vi "Main.vi"() -> ()   [LabVIEW 2026]
doc: "Use this template to build a simple state machine design pattern. Each state executes code and determines which state to transition to."
uses:
  controls/Data.ctl
  controls/State.ctl
panel:
  out "Pos":i32(slide) scale=0.0..250.0
  out "Level 2":bool
  out "Level 1":bool
  out "going up":bool
  out "going down":bool
  out "Up":bool
  out "Down":bool
  in  "Stop":bool
  in  "Up":bool
  in  "Down":bool
  in  "Data":T1
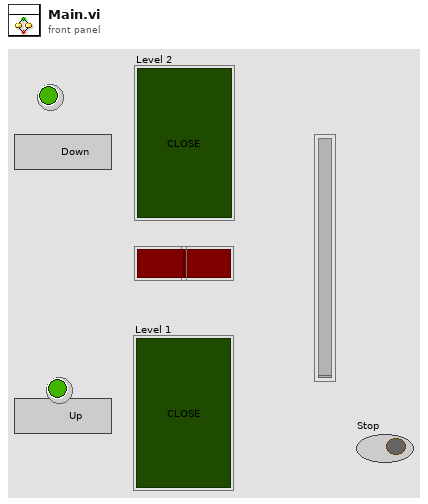
[diagram p1: front panel]
types:
  T1 = typedef "Data.ctl" = cluster{"Level":i32, "Down Pressed":bool, "Up Pressed\n":bool, "Moving Down\n":bool, "Moving Up\n":bool, "L1 Door Open":bool, "L2 Door Open":bool, "Counter":i32, "Previous State":T2, "Pos":i32}
  T2 = typedef "State.ctl" = enum16{"Initialize", "Wait for Event", "Open/Close L1", "Open/Close L2", "Moving Down", "Moving Up", "Exit", ""}
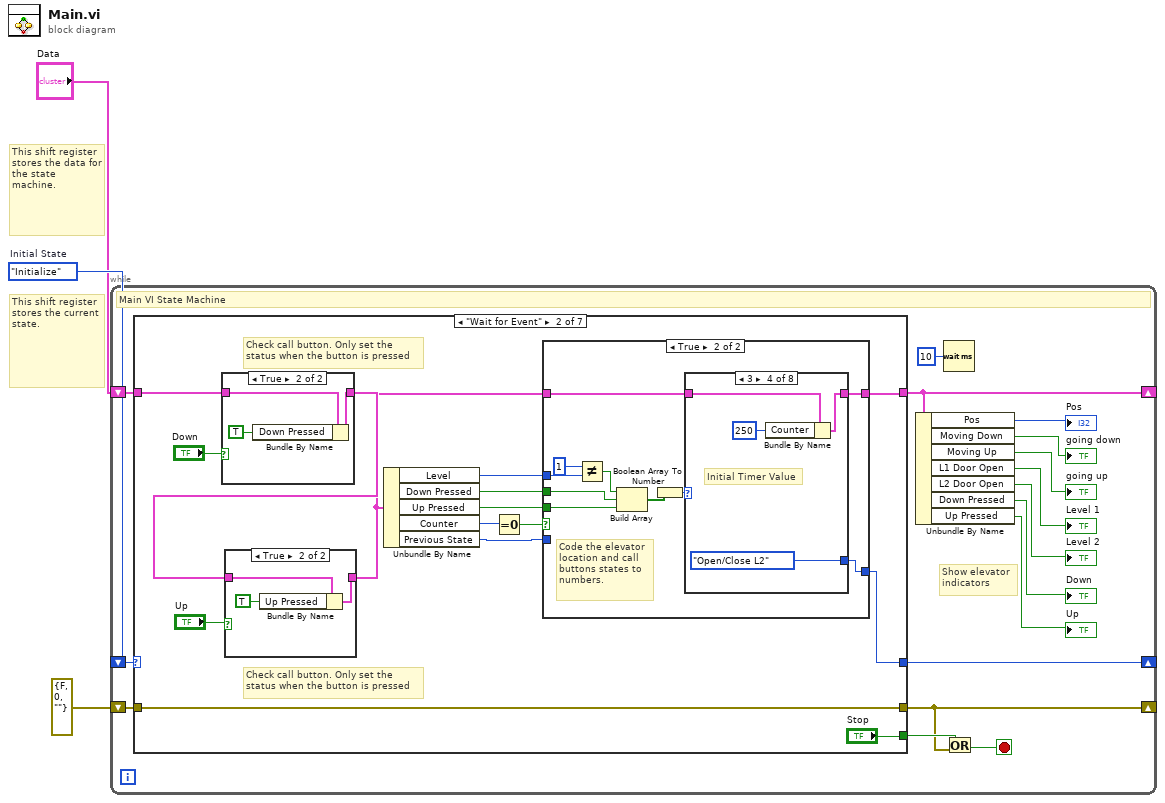
[diagram p0: block diagram]
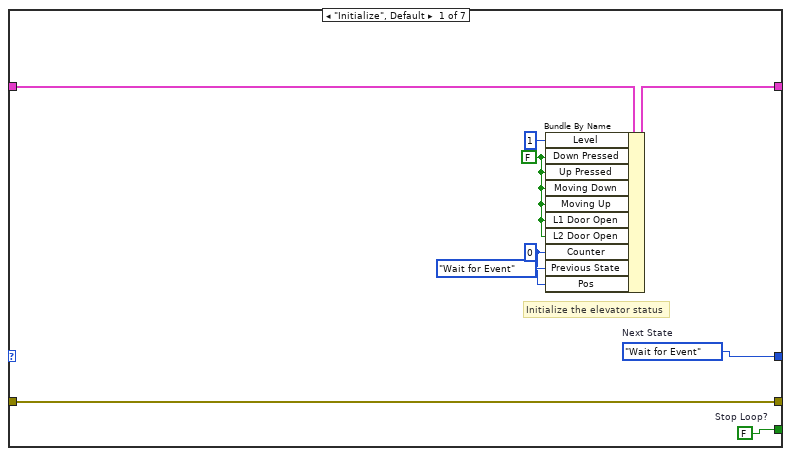
[diagram p2: hidden frame]
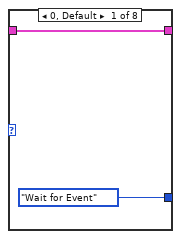
[diagram p4: hidden frame]
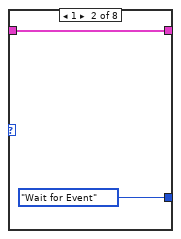
[diagram p5: hidden frame]
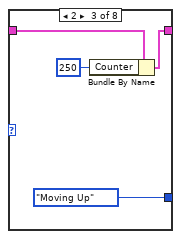
[diagram p6: hidden frame]
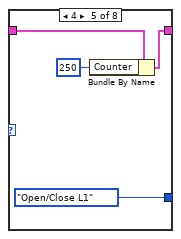
[diagram p7: hidden frame]
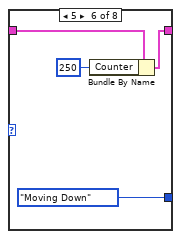
[diagram p8: hidden frame]
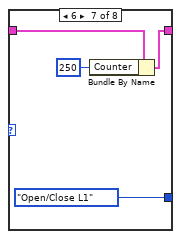
[diagram p9: hidden frame]
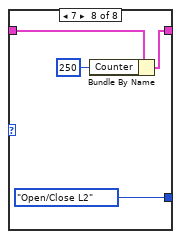
[diagram p10: hidden frame]
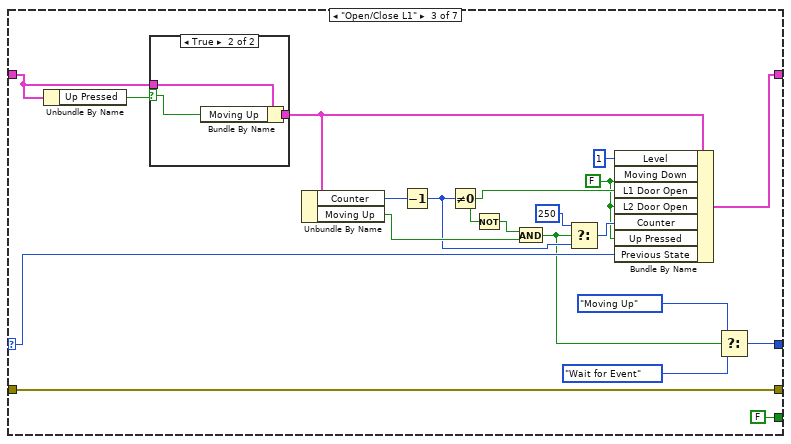
[diagram p13: hidden frame]
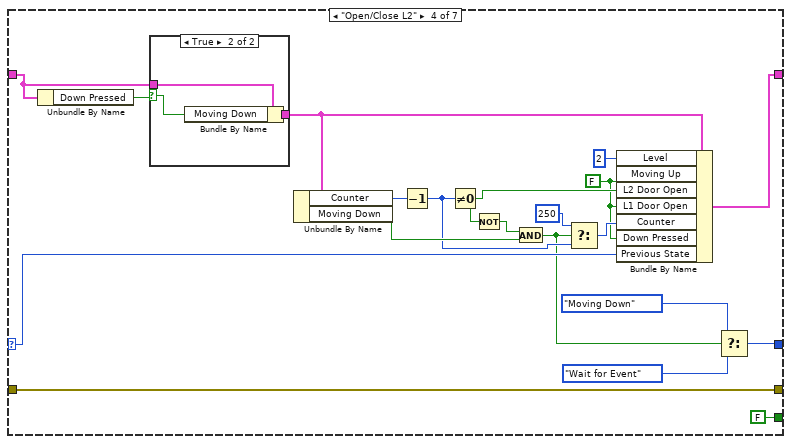
[diagram p15: hidden frame]
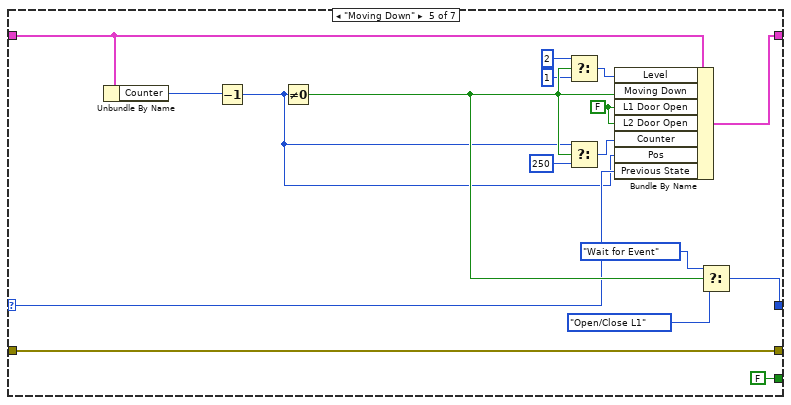
[diagram p17: hidden frame]
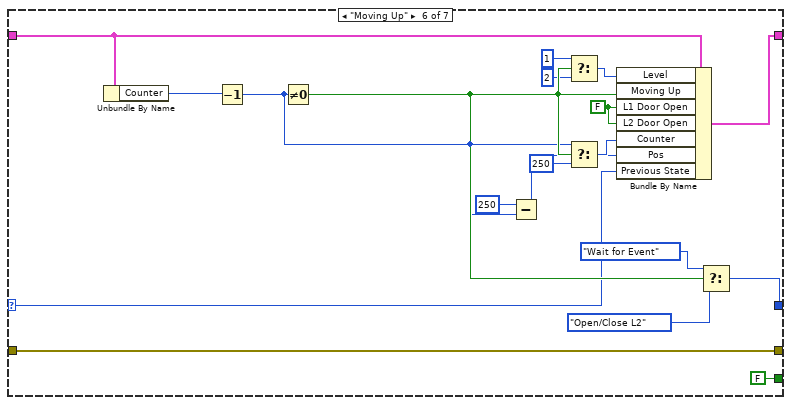
[diagram p18: hidden frame]
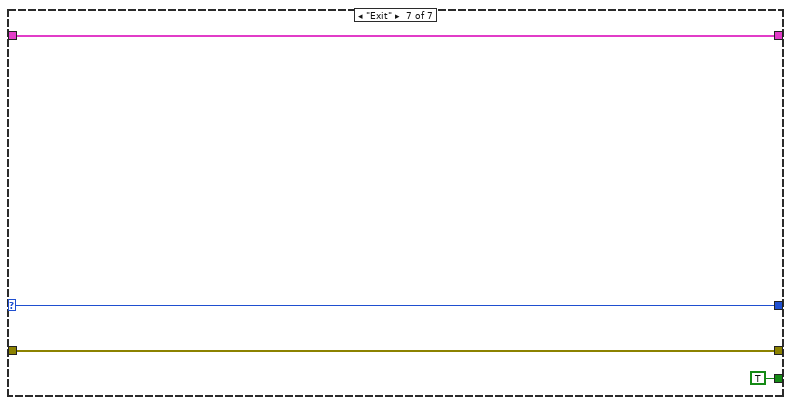
[diagram p19: hidden frame]
diagram:
  w3 = State."Initialize"  # Initial State
  # "This shift register stores the data for the state machine."
  # "This shift register stores the current state."
  n1 = while {
    shift-right: [w4] -> _
    shift-left: w3 -> [w18]
    shift-right: [w14] -> _
    shift-left: "Data" -> [w17]
    shift-right: [w11] -> _
    shift-left: errorcluster {"status"=FALSE, "code"=0, "source"=""} ("error constant") -> [w16]
    stop <- w12 stop-if-true
    # "Show elevator\nindicators"
    # "Main VI State Machine"
    n2 = case shown="\"Wait for Event\"" w18 {
      selector: w18 -> [_ _ w101 w125 w149 w168 w177]
      tunnel: w17 -> [w27 w40 w108 w132 w154 w173 w178]
      tunnel: w16 -> [w28 w43 w111 w135 w156 w175 w179]
      tunnel: [w28 w43 w111 w135 w156 w175 w179] -> w11
      tunnel: [w22 w30 w102 w126 w151 w170 w178] -> w14
      tunnel: [w21 w31 w95 w119 w148 w167 w177] -> w4
      tunnel: [w20 "Stop" FALSE ("Stop") FALSE ("Stop") FALSE ("Stop") FALSE ("Stop") TRUE ("Stop")] -> w15
      frame "Initialize", Default {
        w20 = FALSE  # Stop Loop?
        w21 = State."Wait for Event"  # Next State
        w23 = 0 ("Counter")
        w24 = FALSE ("Down Pressed")
        # "Initialize the elevator status"
        n3 = Bundle By Name(cluster=w27, "Level"=1, "Down Pressed"=w24, "Up Pressed"=w24, "Moving Down"=w24, "Moving Up"=w24, "L1 Door Open"=w24, "L2 Door Open"=w24, "Counter"=w23, "Previous State"=State."Wait for Event", "Pos"=w23) -> (w22:T1)
      }
      frame "Wait for Event" {
        # "Check call button. Only set the\nstatus when the button is pressed"
        # "Check call button. Only set the\nstatus when the button is pressed"
        n4 = case shown="True" "Down" {
          tunnel: w40 -> [w88 w90]
          tunnel: [w88 w89] -> w39
          frame False {
          }
          frame True {
            n5 = Bundle By Name(cluster=w90, "Down Pressed"=TRUE) -> (w89:T1)
          }
        }
        n6 = case shown="True" "Up" {
          tunnel: w39 -> [w84 w87]
          tunnel: [w84 w86] -> w32
          frame False {
          }
          frame True {
            n7 = Bundle By Name(cluster=w87, "Up Pressed"=TRUE) -> (w86:T1)
          }
        }
        n8 = Unbundle By Name(w32) -> ("Level"=w36:i32, "Down Pressed"=w35:bool, "Up Pressed"=w34:bool, "Counter"=w37:i32, "Previous State"=w33:T2)
        n9 = Equal To 0?(x=w37) -> (x = 0?=w38:bool)
        n10 = case shown="True" w38 {
          tunnel: w36 -> [_ w50]
          tunnel: w35 -> [_ w52]
          tunnel: w34 -> [_ w51]
          tunnel: w33 -> [w44 _]
          tunnel: w32 -> [w45 w48]
          tunnel: [w45 w47] -> w30
          tunnel: [w44 w46] -> w31
          frame False {
          }
          frame True {
            # "Code the elevator\nlocation and call\nbuttons states to\nnumbers."
            n11 = Not Equal?(x=1, y=w50) -> (x != y?=w55:bool)
            n12 = Build Array(w55, w52, w51) -> (w54:bool[])
            n13 = Boolean Array To Number(Boolean array=w54) -> (number=w53:u32)
            n14 = case shown="3" w53 {
              tunnel: w48 -> [w57 w59 w62 w66 w70 w74 w78 w82]
              tunnel: [w57 w59 w61 w65 w69 w73 w77 w81] -> w47
              tunnel: [State."Wait for Event" ("Previous State") State."Wait for Event" ("Previous State") State."Moving Up" ("Previous State") State."Open/Close L2" ("Previous State") State."Open/Close L1" ("Previous State") State."Moving Down" ("Previous State") State."Open/Close L1" ("Previous State") State."Open/Close L2" ("Previous State")] -> w46
              frame 0, Default {
              }
              frame 1 {
              }
              frame 2 {
                n15 = Bundle By Name(cluster=w62, "Counter"=250) -> (w61:T1)
              }
              frame 3 {
                # "Initial Timer Value"
                n16 = Bundle By Name(cluster=w66, "Counter"=250) -> (w65:T1)
              }
              frame 4 {
                n17 = Bundle By Name(cluster=w70, "Counter"=250) -> (w69:T1)
              }
              frame 5 {
                n18 = Bundle By Name(cluster=w74, "Counter"=250) -> (w73:T1)
              }
              frame 6 {
                n19 = Bundle By Name(cluster=w78, "Counter"=250) -> (w77:T1)
              }
              frame 7 {
                n20 = Bundle By Name(cluster=w82, "Counter"=250) -> (w81:T1)
              }
            }
          }
        }
      }
      frame "Open/Close L1" {
        w97 = FALSE ("Moving Down")
        n21 = Unbundle By Name(w108) -> ("Up Pressed"=w109:bool)
        n22 = case shown="True" w109 {
          selector: w109 -> [_ w114]
          tunnel: w108 -> [w112 w115]
          tunnel: [w112 w113] -> w103
          frame False {
          }
          frame True {
            n23 = Bundle By Name(cluster=w115, "Moving Up"=w114) -> (w113:T1)
          }
        }
        n24 = Unbundle By Name(w103) -> ("Counter"=w107:i32, "Moving Up"=w106:bool)
        n25 = Decrement(x=w107) -> (x-1=w105:i32)
        n26 = Not Equal To 0?(x=w105) -> (x != 0?=w100:bool)
        n27 = Not(x=w100) -> (.not. x?=w110:bool)
        n28 = And(x=w110, y=w106) -> (x .and. y?=w96:bool)
        n29 = Select(t=250, s=w96, f=w105) -> (s? t:f=w99:i32)
        n30 = Bundle By Name(cluster=w103, "Level"=1, "Moving Down"=w97, "L1 Door Open"=w100, "L2 Door Open"=w97, "Counter"=w99, "Up Pressed"=w97, "Previous State"=w101) -> (w102:T1)
        n31 = Select(t=State."Moving Up" ("Previous State"), s=w96, f=State."Wait for Event" ("Previous State")) -> (s? t:f=w95:T2)
      }
      frame "Open/Close L2" {
        w121 = FALSE ("Moving Down")
        n32 = Unbundle By Name(w132) -> ("Down Pressed"=w133:bool)
        n33 = case shown="True" w133 {
          selector: w133 -> [_ w138]
          tunnel: w132 -> [w136 w139]
          tunnel: [w136 w137] -> w127
          frame False {
          }
          frame True {
            n34 = Bundle By Name(cluster=w139, "Moving Down"=w138) -> (w137:T1)
          }
        }
        n35 = Unbundle By Name(w127) -> ("Counter"=w131:i32, "Moving Down"=w130:bool)
        n36 = Decrement(x=w131) -> (x-1=w129:i32)
        n37 = Not Equal To 0?(x=w129) -> (x != 0?=w124:bool)
        n38 = Not(x=w124) -> (.not. x?=w134:bool)
        n39 = And(x=w134, y=w130) -> (x .and. y?=w120:bool)
        n40 = Select(t=250, s=w120, f=w129) -> (s? t:f=w123:i32)
        n41 = Bundle By Name(cluster=w127, "Level"=2, "Moving Up"=w121, "L2 Door Open"=w124, "L1 Door Open"=w121, "Counter"=w123, "Down Pressed"=w121, "Previous State"=w125) -> (w126:T1)
        n42 = Select(t=State."Moving Down" ("Previous State"), s=w120, f=State."Wait for Event" ("Previous State")) -> (s? t:f=w119:T2)
      }
      frame "Moving Down" {
        w142 = FALSE ("L1 Door Open")
        n43 = Unbundle By Name(w154) -> ("Counter"=w155:i32)
        n44 = Decrement(x=w155) -> (x-1=w140:i32)
        n45 = Not Equal To 0?(x=w140) -> (x != 0?=w150:bool)
        n46 = Select(t=2, s=w150, f=1) -> (s? t:f=w153:i32)
        n47 = Select(t=w140, s=w150, f=250) -> (s? t:f=w152:i32)
        n48 = Bundle By Name(cluster=w154, "Level"=w153, "Moving Down"=w150, "L1 Door Open"=w142, "L2 Door Open"=w142, "Counter"=w152, "Pos"=w140, "Previous State"=w149) -> (w151:T1)
        n49 = Select(t=State."Wait for Event" ("Previous State"), s=w150, f=State."Open/Close L1" ("Previous State")) -> (s? t:f=w148:T2)
      }
      frame "Moving Up" {
        w161 = FALSE ("L1 Door Open")
        n50 = Unbundle By Name(w173) -> ("Counter"=w174:i32)
        n51 = Decrement(x=w174) -> (x-1=w158:i32)
        n52 = Not Equal To 0?(x=w158) -> (x != 0?=w169:bool)
        n53 = Subtract(x=250, y=w158) -> (x-y=w159:i32)
        n54 = Select(t=1, s=w169, f=2) -> (s? t:f=w172:i32)
        n55 = Select(t=w158, s=w169, f=250) -> (s? t:f=w171:i32)
        n56 = Bundle By Name(cluster=w173, "Level"=w172, "Moving Up"=w169, "L1 Door Open"=w161, "L2 Door Open"=w161, "Counter"=w171, "Pos"=w159, "Previous State"=w168) -> (w170:T1)
        n57 = Select(t=State."Wait for Event" ("Previous State"), s=w169, f=State."Open/Close L2" ("Previous State")) -> (s? t:f=w167:T2)
      }
      frame "Exit" {
      }
    }
    n58 = Unbundle By Name(w14) -> ("Pos"=→"Pos":i32, "Moving Down"=→"going down":bool, "Moving Up"=→"going up":bool, "L1 Door Open"=→"Level 1":bool, "L2 Door Open"=→"Level 2":bool, "Down Pressed"=→"Down":bool, "Up Pressed"=→"Up":bool)
    n59 = Wait (ms)(milliseconds to wait=u32 10) -> ()  [unwired: 1 out]
    n60 = Or(x=w15, y=w11) -> (x .or. y?=w12:bool)
  }
